vi "Plant First Order Step.vi"(8 "now ms":dbl, 9 "dt s":dbl=0.1, 10 "Plant Setpoints":T2, 11 "current Plant Feedback":T1) -> (3 "new Plant Feedback":T1)   [LabVIEW 2026]
doc: "One integration step of the simulated VTU plant. Each channel moves toward its setpoint as a first-order lag: x += (sp - x) * (1 - exp(-dt/tau)), with tau 0.8 s for pressure, 0.6 s for flow and 0.3 s for displacement. The new feedback's timestamp_ms is set to now ms. Pure function, no error terminals, AF-free."
uses:
  Typedefs/Plant Feedback.ctl
  Typedefs/Plant Setpoints.ctl
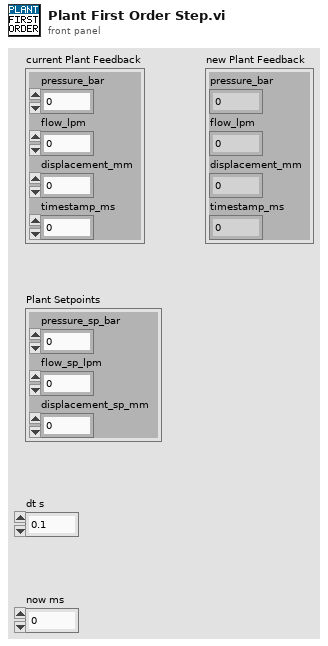
[diagram p1: front panel]
types:
  T1 = typedef "Plant Feedback.ctl" = cluster{"pressure_bar":dbl, "flow_lpm":dbl, "displacement_mm":dbl, "timestamp_ms":dbl}
  T2 = typedef "Plant Setpoints.ctl" = cluster{"pressure_sp_bar":dbl, "flow_sp_lpm":dbl, "displacement_sp_mm":dbl}
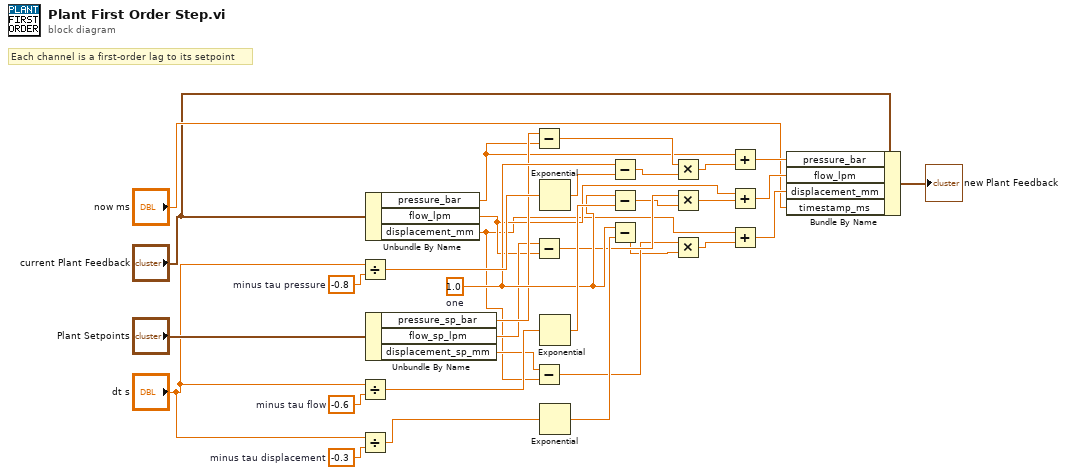
[diagram p0: block diagram]
diagram:
  w23 = 1.0  # one
  w29 = -0.3  # minus tau displacement
  w31 = -0.6  # minus tau flow
  w32 = -0.8  # minus tau pressure
  # "Each channel is a first-order lag to its setpoint"
  n1 = Divide(x="dt s", y=w32) -> (x/y=w28:dbl)
  n2 = Divide(x="dt s", y=w31) -> (x/y=w27:dbl)
  n3 = Divide(x="dt s", y=w29) -> (x/y=w26:dbl)
  n4 = Unbundle By Name("current Plant Feedback") -> ("pressure_bar"=w12:dbl, "flow_lpm"=w10:dbl, "displacement_mm"=w8:dbl)
  n5 = Unbundle By Name("Plant Setpoints") -> ("pressure_sp_bar"=w21:dbl, "flow_sp_lpm"=w20:dbl, "displacement_sp_mm"=w19:dbl)
  n6 = Subtract(x=w21, y=w12) -> (x-y=w18:dbl)
  n7 = Subtract(x=w20, y=w10) -> (x-y=w16:dbl)
  n8 = Subtract(x=w19, y=w8) -> (x-y=w14:dbl)
  n9 = Exponential(1:w28) -> (0:w25:dbl)
  n10 = Exponential(1:w27) -> (0:w24:dbl)
  n11 = Exponential(1:w26) -> (0:w22:dbl)
  n12 = Subtract(x=w23, y=w25) -> (x-y=w17:dbl)
  n13 = Subtract(x=w23, y=w24) -> (x-y=w15:dbl)
  n14 = Subtract(x=w23, y=w22) -> (x-y=w13:dbl)
  n15 = Multiply(x=w18, y=w17) -> (x*y=w11:dbl)
  n16 = Multiply(x=w16, y=w15) -> (x*y=w9:dbl)
  n17 = Multiply(x=w14, y=w13) -> (x*y=w7:dbl)
  n18 = Add(x=w12, y=w11) -> (x+y=w6:dbl)
  n19 = Add(x=w10, y=w9) -> (x+y=w5:dbl)
  n20 = Add(x=w8, y=w7) -> (x+y=w4:dbl)
  n21 = Bundle By Name(cluster="current Plant Feedback", "pressure_bar"=w6, "flow_lpm"=w5, "displacement_mm"=w4, "timestamp_ms"="now ms") -> (→"new Plant Feedback":T1)
